vi "CP profie graph.vi"(11 "Assigned CP Profile plus":T1) -> (3 "CP Graph Profile":cluster{i32[], dbl[]}[](graph))   [LabVIEW 2018]
panel:
  in  "Assigned CP Profile":T2
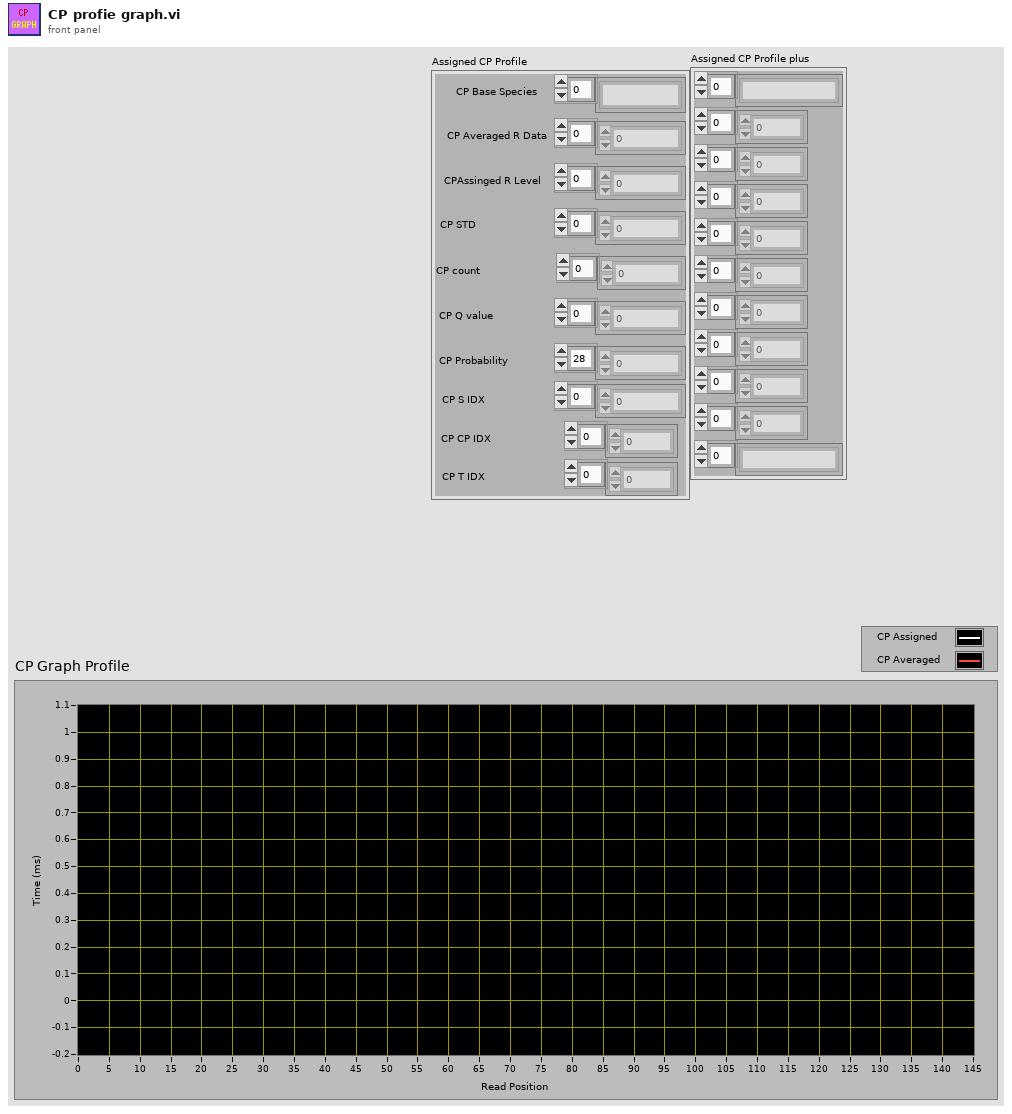
[diagram p1: front panel]
types:
  T1 = cluster{string[], dbl[], dbl[], dbl[], i32[], dbl[], dbl[], i32[], i32[], i32[], string[]}
  T2 = cluster{"CP Base Species":string[], "CP Averaged R Data":dbl[], "CPAssinged R Level":dbl[], "CP STD":dbl[], "CP count":i32[], "CP Q value":dbl[], "CP Probability":dbl[], "CP S IDX":i32[], "CP CP IDX":i32[], "CP T IDX":i32[]}
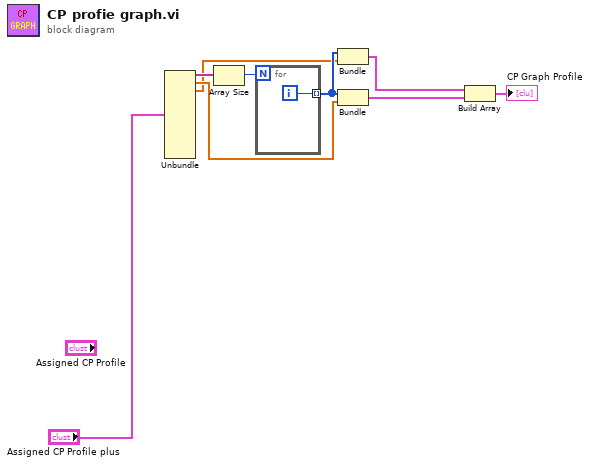
[diagram p0: block diagram]
diagram:
  n1 = Unbundle("Assigned CP Profile plus") -> (w9:string[], w6:dbl[], w5:dbl[])  [unwired: 8 out]
  n2 = Array Size(array=w9) -> (size(s)=w8:i32)
  n3 = for {
    N: w8 -> [_]
    tunnel: [w10] -> w7 mode=indexing
    i -> [w10]
  }
  n4 = Bundle(w7, w5) -> (w3:cluster{i32[], dbl[]})  [unwired: 1 in]
  n5 = Bundle(w7, w6) -> (w2:cluster{i32[], dbl[]})  [unwired: 1 in]
  n6 = Build Array(w3, w2) -> (→"CP Graph Profile":cluster{i32[], dbl[]}[])
